vi "Call.vi"(8 "error in (no error)":errorcluster, 9 "Arguments":variant, 10 "Function":string, 11 "Tool in":refnum<class "MockTool.lvclass">) -> (0 "error out":errorcluster, 2 "Result":variant, 3 "Tool out":refnum<class "MockTool.lvclass">)   [LabVIEW 2017, in "MockTool.lvclass"]
uses:
  MockTool.lvclass
  <vilib>/LVH/i3 JSON/JSON Parsing/Get Object Parameter Files/Get Object Parameter - Numeric.vi
  <vilib>/LVH/i3 JSON/JSON Generation/Create Value Files/Create Value - Object.vi
  <vilib>/LVH/i3 JSON/JSON Generation/Add Object Parameter Files/Add Object Parameter - Numeric.vi
  <vilib>/LVH/i3 JSON/i3-json.lvlib
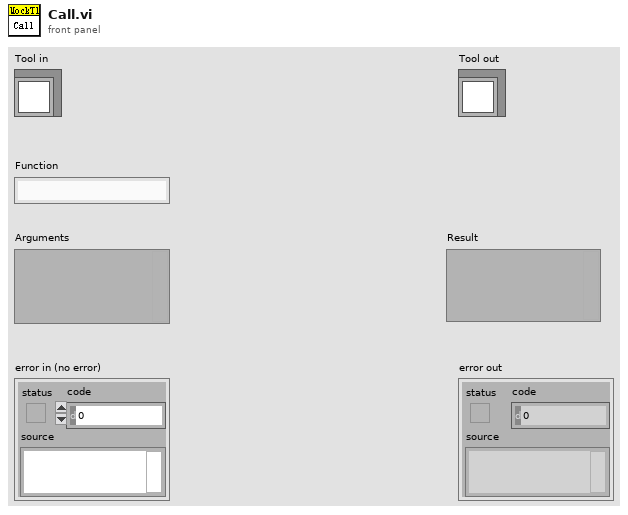
[diagram p1: front panel]
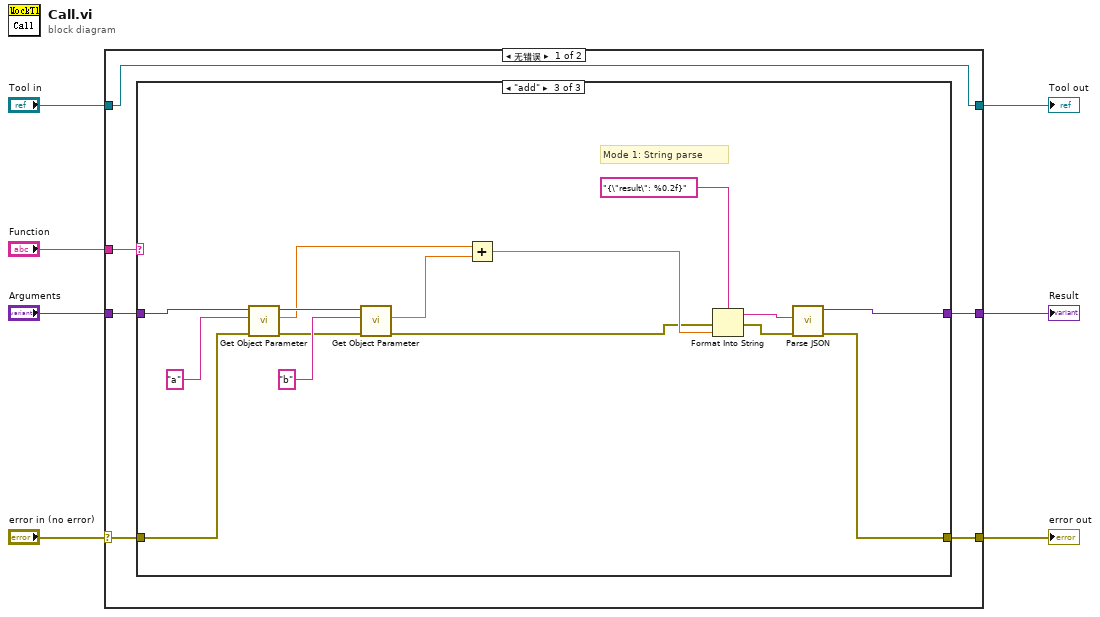
[diagram p0: block diagram]
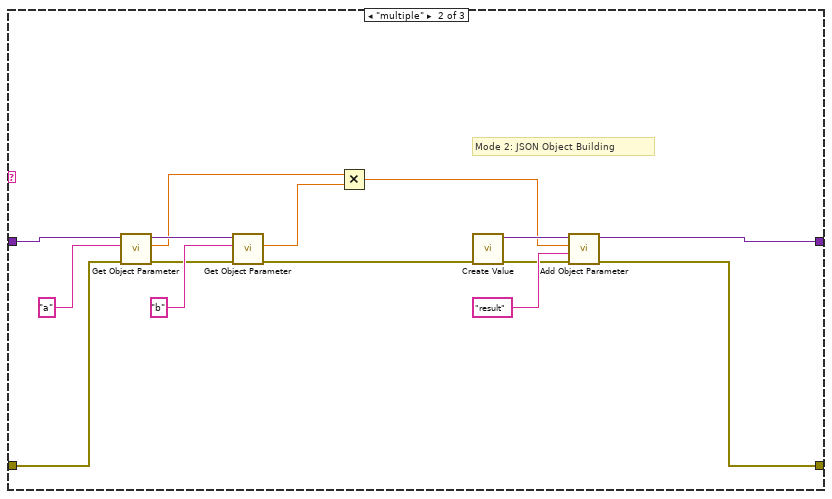
[diagram p3: hidden frame]
diagram:
  n1 = case shown="无错误" "error in (no error)" {
    selector: "error in (no error)" -> [w10 w48]
    tunnel: [w11 w48] -> w1
    tunnel: "Function" -> [w13 _]
    tunnel: "Arguments" -> [w12 w47]
    tunnel: [w9 w47] -> w2
    tunnel: "Tool in" -> [w8 w46]
    tunnel: [w8 w46] -> w3
    frame No Error {
      n2 = case shown="\"add\"" w13 {
        tunnel: w12 -> [w14 w24 w45]
        tunnel: [w15 w16 w34] -> w11
        tunnel: w10 -> [w15 w23 w35]
        tunnel: [w14 w17 w36] -> w9
        frame "", Default {
        }
        frame "multiple" {
          # "Mode 2: JSON Object Building"
          n3 = call-poly <vilib>:"Get Object Parameter.vi"("error in (no error)"=w23, "Parameter Name"="a", "JSON Tree In (JSON Object)"=w24) -> ("error out"=w27:errorcluster, "Double Value"=w26:dbl, "JSON Tree Out Passthrough"=w28:variant)  [unwired: 5 in, 1 out]
          n4 = call-poly <vilib>:"Get Object Parameter.vi"("error in (no error)"=w27, "Parameter Name"="b", "JSON Tree In (JSON Object)"=w28) -> ("error out"=w20:errorcluster, "Double Value"=w25:dbl)  [unwired: 5 in, 2 out]
          n5 = Multiply(x=w26, y=w25) -> (x*y=w18:dbl)
          n6 = call-poly <vilib>:"Create Value.vi"("error in (no error)"=w20) -> ("error out"=w19:errorcluster, "JSON Tree"=w22:variant)  [unwired: 9 in]
          n7 = call-poly <vilib>:"Add Object Parameter.vi"("error in (no error)"=w19, "Name"="result", "Numeric"=w18, "JSON Tree in (JSON Object)"=w22) -> ("error out"=w16:errorcluster, "JSON Tree out (JSON Object)"=w17:variant)  [unwired: 6 in]
        }
        frame "add" {
          # "Mode 1: String parse"
          n8 = call-poly <vilib>:"Get Object Parameter.vi"("error in (no error)"=w35, "Parameter Name"="a", "JSON Tree In (JSON Object)"=w45) -> ("error out"=w41:errorcluster, "Double Value"=w40:dbl, "JSON Tree Out Passthrough"=w42:variant)  [unwired: 5 in, 1 out]
          n9 = call-poly <vilib>:"Get Object Parameter.vi"("error in (no error)"=w41, "Parameter Name"="b", "JSON Tree In (JSON Object)"=w42) -> ("error out"=w33:errorcluster, "Double Value"=w39:dbl)  [unwired: 5 in, 2 out]
          n10 = Add(x=w40, y=w39) -> (x+y=w38:dbl)
          n11 = Format Into String(format string="{\"result\": %0.2f}" ("格式字符串"), error in=w33, w38) -> (resulting string=w37:string, error out=w32:errorcluster)  [unwired: 1 in]
          n12 = call <vilib>:"Parse JSON.vi"("error in (no error)"=w32, "JSON String"=w37) -> ("error out"=w34:errorcluster, "JSON Tree"=w36:variant)  [unwired: 6 in, 2 out]
        }
      }
    }
    frame Error {
    }
  }
  "Tool out" <- w3
  "error out" <- w1
  "Result" <- w2
